vi "RDV-addDataToGraph-data.vi"(8 "error in (no error)":errorcluster, 11 "RDV-Reflection_Data_viewer in":refnum<class "RDV-Reflection_Data_viewer.lvclass">) -> (0 "error out":errorcluster, 3 "RDV-Reflection_Data_viewer out":refnum<class "RDV-Reflection_Data_viewer.lvclass">)   [LabVIEW 2020, in "RDV-Reflection_Data_viewer.lvclass"]
doc: "Writes the data in the viewer's map to the graphs."
uses:
  RDV-Reflection_Data_viewer.lvclass
  RDV-Reflection_Data_viewer.lvclass/RDV-Reflection_Data_viewer.ctl
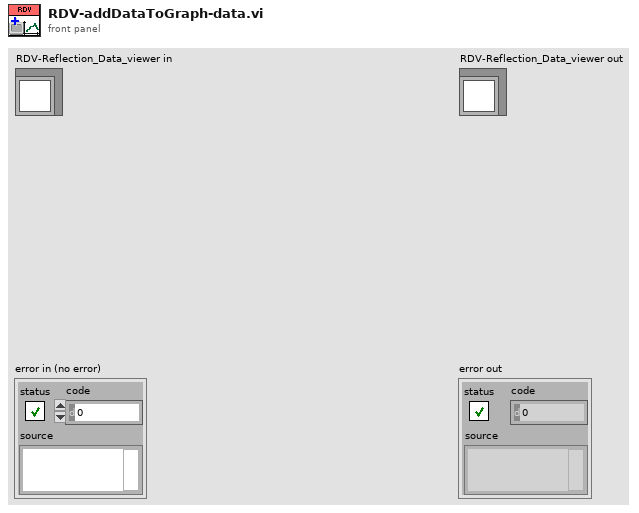
[diagram p1: front panel]
types:
  T1 = cluster{"Frequency":dbl[], "Reflection'":dbl[]}[]
  T2 = cluster{"Frequency":dbl[], "Reflection'":dbl[]}[][]
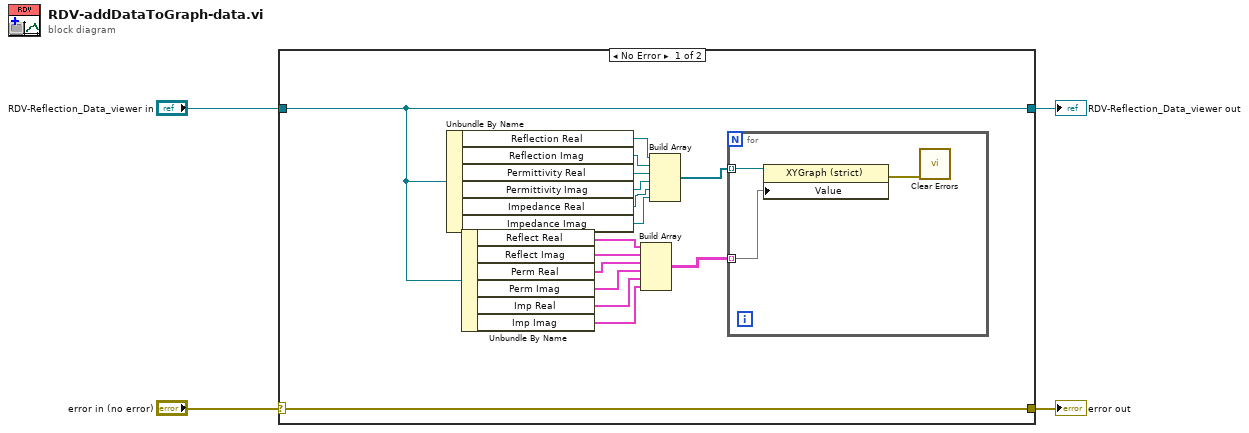
[diagram p0: block diagram]
diagram:
  n1 = case shown="No Error" "error in (no error)" {
    selector: "error in (no error)" -> [w20 w25]
    tunnel: [w20 w25] -> w3
    tunnel: [w15 w24] -> w1
    tunnel: "RDV-Reflection_Data_viewer in" -> [w15 w24]
    frame No Error {
      n2 = Unbundle By Name(w15) -> ("Reflection Real"=w14:refnum<vi>, "Reflection Imag"=w13:refnum<vi>, "Permittivity Real"=w12:refnum<vi>, "Permittivity Imag"=w11:refnum<vi>, "Impedance Real"=w8:refnum<vi>, "Impedance Imag"=w7:refnum<vi>)
      n3 = Unbundle By Name(w15) -> ("Reflect Real"=w19:T1, "Reflect Imag"=w18:T1, "Perm Real"=w17:T1, "Perm Imag"=w16:T1, "Imp Real"=w6:T1, "Imp Imag"=w5:T1)
      n4 = Build Array(w19, w18, w17, w16, w6, w5) -> (w9:T2)
      n5 = Build Array(w14, w13, w12, w11, w8, w7) -> (w10:refnum<vi>[])
      n6 = for {
        tunnel: w10 -> [w23] mode=indexing
        tunnel: w9 -> [w22] mode=indexing
        n7 = property on="Property Node" class="XYGraph (strict)"(reference=w23, "Value"=w22) -> (error out=w21:errorcluster)  [unwired: 1 in, 1 out]
        n8 = call <vilib>:"Clear Errors.vi"("error in (no error)"=w21) -> ()  [unwired: 5 in, 2 out]
      }
    }
    frame Error {
    }
  }
  "error out" <- w3
  "RDV-Reflection_Data_viewer out" <- w1
